vi "ToolReturnToJsonRpcResponseCluster.vi"(8 "error in (no error)":errorcluster, 10 "ToolReturn":cluster{"id":string, "result":variant}) -> (0 "error out":errorcluster, 2 "JsonRPCHttpResponseBody":T1)   [LabVIEW 2017]
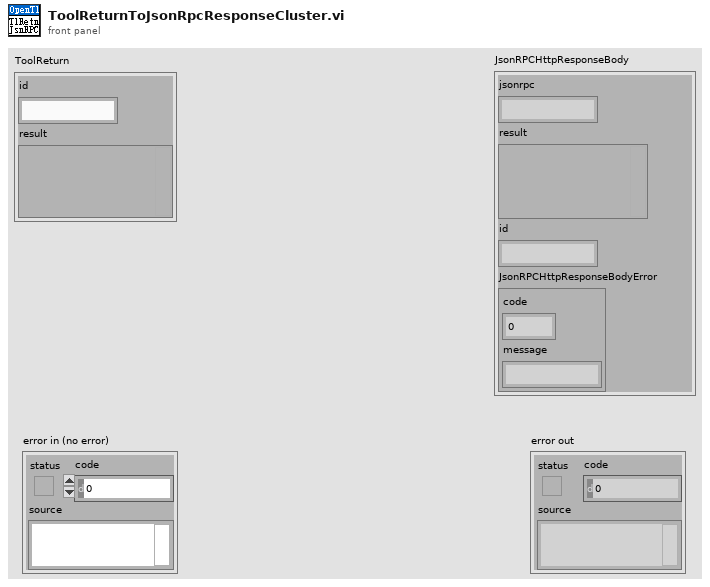
[diagram p1: front panel]
types:
  T1 = cluster{"jsonrpc":string, "result":variant, "id":string, "JsonRPCHttpResponseBodyError":cluster{"code":i32, "message":string}}
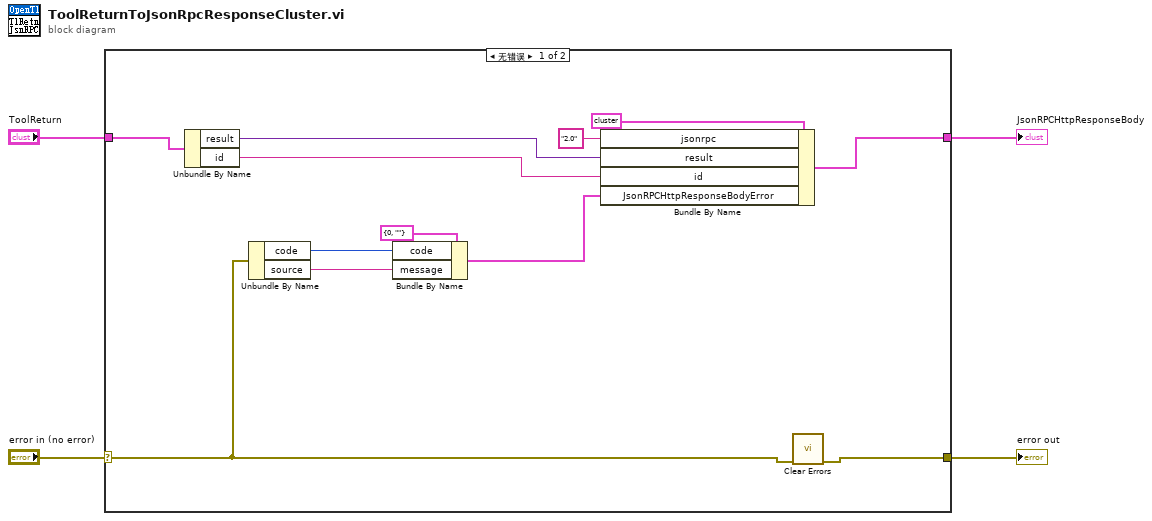
[diagram p0: block diagram]
diagram:
  n1 = case shown="无错误" "error in (no error)" {
    selector: "error in (no error)" -> [w7 w17]
    tunnel: [w6 w17] -> w3
    tunnel: "ToolReturn" -> [w15 _]
    tunnel: [w5 _] -> w1
    frame No Error {
      n2 = Unbundle By Name(w15) -> ("result"=w13:variant, "id"=w12:string)
      n3 = Unbundle By Name(w7) -> ("code"=w10:i32, "source"=w9:string)
      n4 = Bundle By Name(cluster=cluster{"code":i32, "message":string} {"code"=0, "message"=""} ("JsonRPCHttpResponseBodyError"), "code"=w10, "message"=w9) -> (w8:cluster{"code":i32, "message":string})
      n5 = Bundle By Name(cluster=T1 {"jsonrpc"="", "result"=variant, "id"="", "JsonRPCHttpResponseBodyError"={"code"=0, "message"=""}} ("JsonRPCHttpResponseBody"), "jsonrpc"="2.0", "result"=w13, "id"=w12, "JsonRPCHttpResponseBodyError"=w8) -> (w5:T1)
      n6 = call <vilib>:"Clear Errors.vi"("error in (no error)"=w7) -> ("error out"=w6:errorcluster)  [unwired: 5 in, 1 out]
    }
    frame Error {
    }
  }
  "error out" <- w3
  "JsonRPCHttpResponseBody" <- w1
